vi "Edit Channel--Dialog.vi"(8 "error in (no error)":errorcluster, 10 "Channels":string[](array[string]), 11 "ChannelManagerUI in":refnum<class "ChannelManagerUI.lvclass">) -> (0 "error out":errorcluster, 1 "OK":bool, 2 "Class":refnum<class "Channel.lvclass">, 3 "ChannelManagerUI out":refnum<class "ChannelManagerUI.lvclass">)   [LabVIEW 2021, in "Channel.lvlib" / "ChannelManagerUI.lvlib" / "ChannelManagerUI.lvclass"]
uses:
  ChannelManagerUI.lvclass
  Channel_class/Channel.lvclass
  ChannelManagerUI.lvclass/ChannelManagerUI.ctl
  Configuration_class/Configuration.lvclass
  Channel.lvlib
panel:
  in  "Channel Type":string
  out "Valid?":bool
  in  "Channel Name":string
  in  "OK Button":bool
  in  "Cancel Button":bool
  in  "Specific Channel":string(combo)
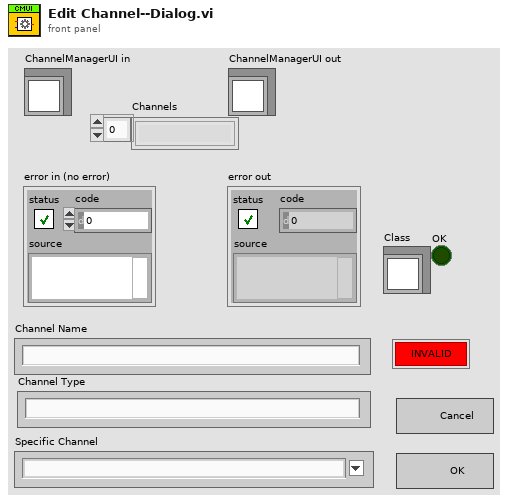
[diagram p1: front panel]
types:
  T1 = enum8{"Enabled", "Disabled", "Disabled and Grayed Out"}
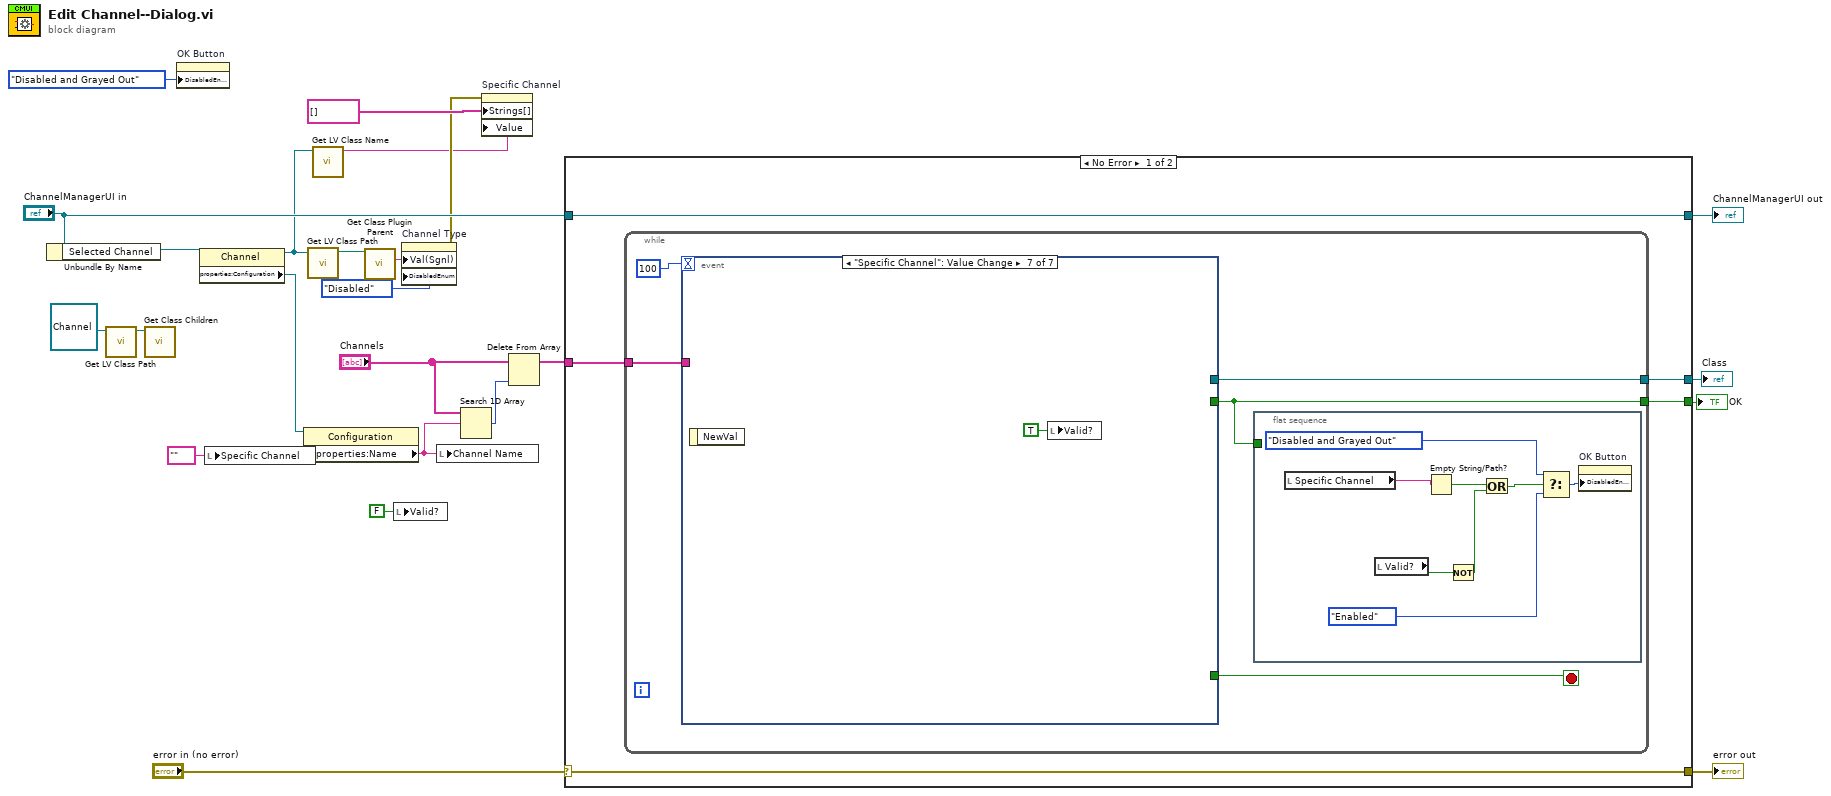
[diagram p0: block diagram]
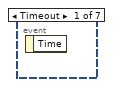
[diagram p2: hidden frame]
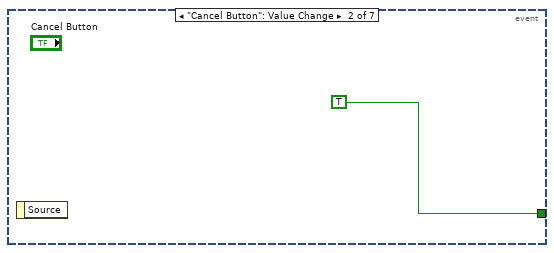
[diagram p3: hidden frame]
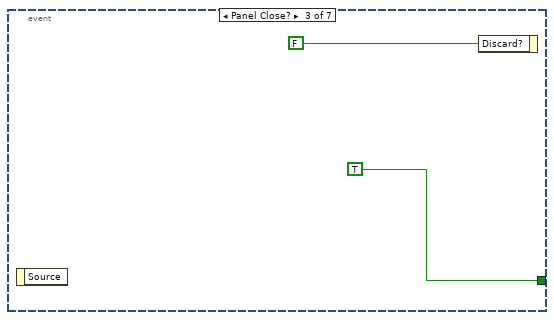
[diagram p4: hidden frame]
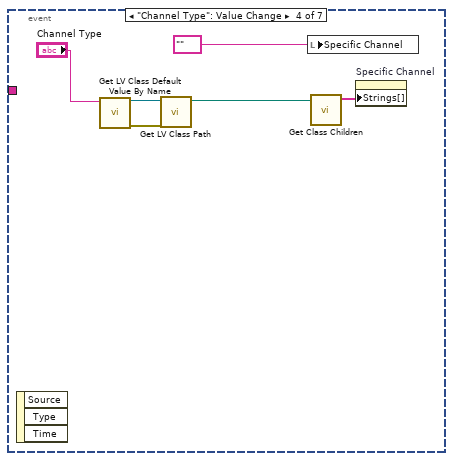
[diagram p5: hidden frame]
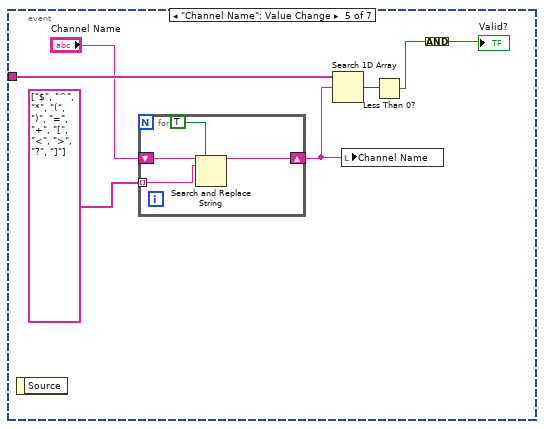
[diagram p6: hidden frame]
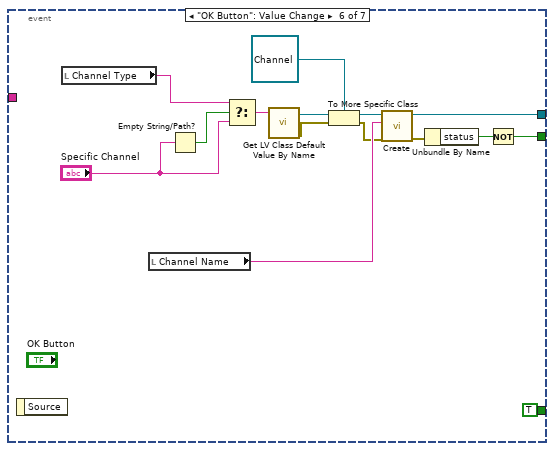
[diagram p7: hidden frame]
diagram:
  n1 = Unbundle By Name("ChannelManagerUI in") -> ("Selected Channel"=w12:refnum<class "Channel.lvclass">)
  n2 = call <vilib>:"Get LV Class Path.vi"("object"=refnum<class "Channel.lvclass"> refnum ("Channel.lvlib:Channel")) -> ("class path"=w20:path)  [unwired: 9 in, 1 out]
  n3 = call "Get Class Children.vi"("LV Class Path"=w20) -> ()  [unwired: 8 in, 3 out]
  n4 = property on="OK Button" class="Bool"("DisabledEnum"=T1."Disabled and Grayed Out" ("Disabled")) -> ()  [unwired: 2 in, 2 out]
  n5 = property class="Channel"(reference=w12) -> (reference out=w7:refnum<class "Channel.lvclass">, "properties:Configuration"=w9:refnum<class "Configuration.lvclass">)  [unwired: 1 in, 1 out]
  n6 = local write "Specific Channel"("" ("Specific Channel")) -> ()
  n7 = property class="Configuration"(reference=w9) -> ("properties:Name"=w4:string)  [unwired: 1 in, 2 out]
  n8 = call <vilib>:"Get LV Class Path.vi"("object"=w7) -> ("class path"=w11:path)  [unwired: 9 in, 1 out]
  n9 = call <vilib>:"Get LV Class Name.vi"("object"=w7) -> ("class name"=w6:string)  [unwired: 9 in, 1 out]
  n10 = call "Get Class Plugin Parent.vi"("LV Class Path"=w11) -> ("Qualified Name"=w10:string)  [unwired: 7 in, 3 out]
  n11 = local write "Valid?"(FALSE ("Valid?")) -> ()
  n12 = property on="Channel Type" class="Str"("Val(Sgnl)"=w10, "DisabledEnum"=T1."Disabled" ("Disabled")) -> (error out=w8:errorcluster)  [unwired: 2 in, 1 out]
  n13 = local write "Channel Name"(w4) -> ()
  n14 = Search 1D Array(1D array="Channels", element=w4) -> (index of element=w2:i32)  [unwired: 1 in]
  n15 = property on="Specific Channel" class="CmbBox"(error in=w8, "Strings[]"=string[] [] ("Strings []"), "Value"=w6) -> ()  [unwired: 1 in, 2 out]
  n16 = Delete From Array(array="Channels", index=w2) -> (array with subset deleted=w1:string[])  [unwired: 1 in, 1 out]
  n17 = case shown="No Error" "error in (no error)" {
    selector: "error in (no error)" -> [w28 w80]
    tunnel: [w28 w80] -> w23
    tunnel: [w29 w79] -> w22
    tunnel: "ChannelManagerUI in" -> [w29 w79]
    tunnel: w1 -> [w27 _]
    tunnel: [w26 _] -> w15
    tunnel: [w25 _] -> w14
    frame No Error {
      n18 = while {
        tunnel: w27 -> [w32]
        tunnel: [w31] -> w26
        tunnel: [w30] -> w25
        stop <- w33 stop-if-true
        n19 = event shown="[6] \"Specific Channel\": Value Change" {
          selector: _ -> [_ _ _ _ _ _ _]
          dyn-events: _ -> [_ _ _ _ _ _ _]
          timeout: 100 -> [_ _ _ _ _ _ _]
          tunnel: [_ TRUE TRUE _ _ TRUE _] -> w33
          tunnel: w32 -> [_ _ _ _ w58 _ _]
          tunnel: [_ _ _ _ _ w66 _] -> w31
          tunnel: [_ _ _ _ _ w65 _] -> w30
          event Timeout {
            n20 = event-data() -> ()  [unwired: 1 in, 1 out]
          }
          event "Cancel Button": Value Change {
            n21 = event-data() -> ()  [unwired: 1 in, 1 out]
          }
          event Panel Close? {
            n22 = event-data() -> ()  [unwired: 1 in, 1 out]
            n23 = event-data("Discard?"=FALSE) -> ()  [unwired: 1 in, 1 out]
          }
          event "Channel Type": Value Change {
            n24 = event-data() -> ()  [unwired: 1 in, 3 out]
            n25 = call <vilib>:"Get LV Class Default Value By Name.vi"("class name"="Channel Type") -> ("error out"=w50:errorcluster, "object"=w51:refnum<class>)  [unwired: 9 in]
            n26 = call <vilib>:"Get LV Class Path.vi"("error in (no error)"=w50, "object"=w51) -> ("class path"=w49:path)  [unwired: 8 in, 1 out]
            n27 = local write "Specific Channel"("" ("Specific Channel")) -> ()
            n28 = call "Get Class Children.vi"("LV Class Path"=w49) -> ("Names"=w48:string[])  [unwired: 8 in, 2 out]
            n29 = property on="Specific Channel" class="CmbBox"("Strings[]"=w48) -> ()  [unwired: 2 in, 2 out]
          }
          event "Channel Name": Value Change {
            n30 = event-data() -> ()  [unwired: 1 in, 1 out]
            n31 = for {
              shift-right: [w61] -> w52
              shift-left: "Channel Name" -> [w62]
              tunnel: string[] ["$", "^", "*", "(", ")", "=", "+", "[", "<", ">", "?", "]"] -> [w59] mode=indexing
              n32 = Search and Replace String(replace all?=TRUE ("replace all? (F)"), input string=w62, search string=w59) -> (result string=w61:string)  [unwired: 5 in, 3 out]
            }
            n33 = Search 1D Array(1D array=w58, element=w52) -> (index of element=w56:i32)  [unwired: 1 in]
            n34 = local write "Channel Name"(w52) -> ()
            n35 = Less Than 0?(x=w56) -> (x < 0?=w55:bool)
            n36 = Compound Arithmetic op=AND(w55) -> (→"Valid?":bool)
          }
          event "OK Button": Value Change {
            n37 = event-data() -> ()  [unwired: 1 in, 1 out]
            n38 = local read "Channel Type"() -> (w63:string)
            n39 = local read "Channel Name"() -> (w71:string)
            n40 = Empty String/Path?(string/path="Specific Channel") -> (empty?=w77:bool)
            n41 = Select(t=w63, s=w77, f="Specific Channel") -> (s? t:f=w76:string)
            n42 = call <vilib>:"Get LV Class Default Value By Name.vi"("class name"=w76) -> ("error out"=w70:errorcluster, "object"=w74:refnum<class>)  [unwired: 9 in]
            n43 = To More Specific Class(target class=refnum<class "Channel.lvclass"> refnum ("Channel.lvlib:Channel"), reference=w74, error in=w70) -> (specific class reference=w72:refnum<class "Channel.lvclass">, error out=w69:errorcluster)
            n44 = call-dynamic "Create.vi"("error in (no error)"=w69, "Name"=w71, "object in"=w72) -> ("error out"=w68:errorcluster, "object out"=w66:refnum<class "Channel.lvclass">)  [unwired: 7 in]
            n45 = Unbundle By Name(w68) -> ("status"=w67:bool)
            n46 = Not(x=w67) -> (.not. x?=w65:bool)
          }
          event "Specific Channel": Value Change {
            n47 = event-data() -> ()  [unwired: 1 in, 1 out]
            n48 = local write "Valid?"(TRUE ("Valid?")) -> ()
          }
        }
        n49 = flat-sequence {
          tunnel: w30 -> [_]
          frame #0 {
            n50 = local read "Specific Channel"() -> (w42:string)
            n51 = local read "Valid?"() -> (w39:bool)
            n52 = Empty String/Path?(string/path=w42) -> (empty?=w38:bool)
            n53 = Not(x=w39) -> (.not. x?=w41:bool)
            n54 = Or(x=w38, y=w41) -> (x .or. y?=w40:bool)
            n55 = Select(t=T1."Disabled and Grayed Out" ("Disabled"), s=w40, f=T1."Enabled") -> (s? t:f=w37:T1)
            n56 = property on="OK Button" class="Bool"("DisabledEnum"=w37) -> ()  [unwired: 2 in, 2 out]
          }
        }
      }
    }
    frame Error {
    }
  }
  "error out" <- w23
  "ChannelManagerUI out" <- w22
  "Class" <- w15
  "OK" <- w14
